vi "Configure Module.vi"(8 "error in (no error)":errorcluster, 10 "IOV ref in":variant, 11 "9224 in":refnum<class "9224.lvclass">) -> (0 "error out":errorcluster, 2 "IOV ref out":variant, 3 "9224 out":refnum<class "9224.lvclass">)   [LabVIEW 2020, in "Modules.lvlib" / "9224.lvclass"]
uses:
  9224.lvclass
  <resource>/objmgr/cRIO.rc
  RSI Module/RSI Module.lvclass
  C:/Users/nitest/Desktop/Git 2020/niveristand-scan-engine-module-libraries/Source/RSI Module/RSI Module.lvclass
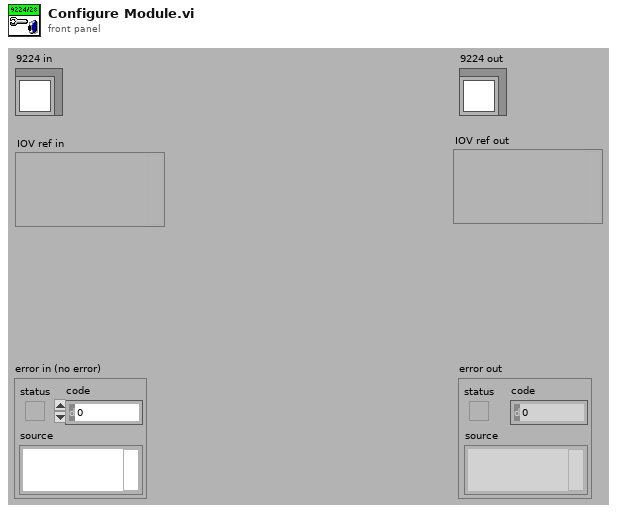
[diagram p1: front panel]
types:
  T1 = typedef "Modules.lvlib/9224.lvclass/Conversion Time.ctl" = u16
  T2 = typedef "Modules.lvlib/RSI Module.lvclass/Module Models.ctl" = enum16{"Empty", "NI 9201", "NI 9203", "NI 9205", "NI 9206", "NI 9207", "NI 9208", "NI 9209", "NI 9210", "NI 9211", "NI 9212", "NI 9213", "NI 9214", "NI 9215", "NI 9216", "NI 9217", "NI 9219", "NI 9220", "NI 9221", "NI 9222", "NI 9223", "NI 9224", "NI 9225", "NI 9226", "NI 9227", "NI 9228", "NI 9229", "NI 9233", "NI 9234", "NI 9235", "NI 9236", "NI 9237", "NI 9239", "NI 9242", "NI 9244", "NI 9253", "NI 9263", "NI 9264", "NI 9265", "NI 9266", "NI 9269", "NI 9344", "NI 9350", "NI 9375", "NI 9401", "NI 9402", "NI 9403", "NI 9411", "NI 9421", "NI 9422", "NI 9423", "NI 9425", "NI 9426", "NI 9435", "NI 9436", "NI 9437", "NI 9472", "NI 9474", "NI 9475", "NI 9476", "NI 9477", "NI 9478", "NI 9481", "NI 9482", "NI 9485"}
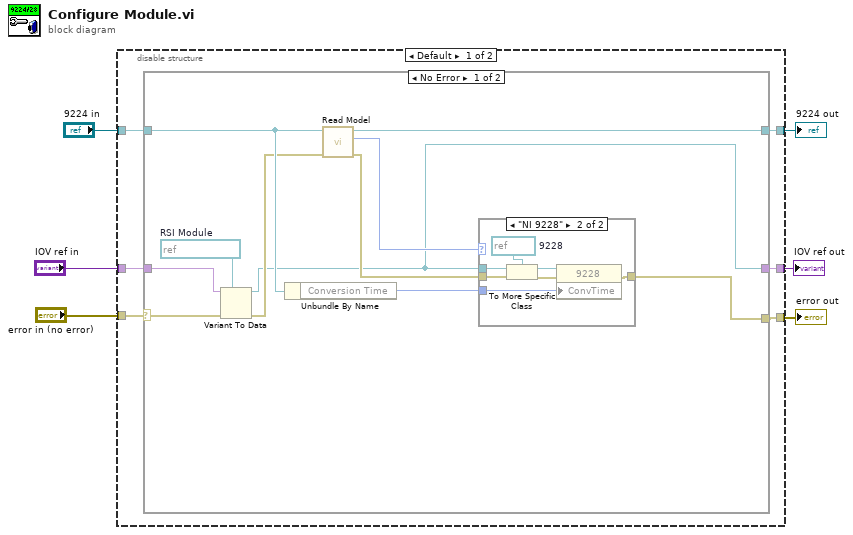
[diagram p0: block diagram]
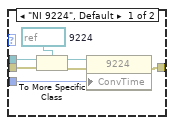
[diagram p2: hidden frame]
diagram:
  n1 = disable-structure shown="Default" {
    disable-tunnel: "9224 in" -> [w12 w43]
    disable-tunnel: "IOV ref in" -> [w11 w42]
    disable-tunnel: "error in (no error)" -> [w10 w41]
    disable-tunnel: [w9 w41] -> w3
    disable-tunnel: [w8 w42] -> w2
    disable-tunnel: [w7 w43] -> w1
    frame condition #0 {
      n2 = case shown="No Error" w10 {
        selector: w10 -> [w22 w40]
        tunnel: [w17 w40] -> w9
        tunnel: [w23 w39] -> w7
        tunnel: w12 -> [w21 w39]
        tunnel: w11 -> [w15 w38]
        tunnel: [w14 w38] -> w8
        frame No Error {
          w13 = refnum<k21> refnum  # RSI Module
          n3 = Variant To Data(error in=w22, type=w13, Variant=w15) -> (data=w14:refnum<k21>, error out=w16:errorcluster)
          n4 = Unbundle By Name(w21) -> ("Conversion Time"=w18:T1)
          n5 = call "Read Model.vi"("error in (no error)"=w16, "RSI Module in"=w21) -> ("error out"=w19:errorcluster, "Model"=w20:T2, "RSI Module out"=w23:refnum<class "9224.lvclass">)  [unwired: 7 in]
          n6 = case shown="\"NI 9228\"" w20 {
            tunnel: w19 -> [w30 w31]
            tunnel: [w26 w32] -> w17
            tunnel: w14 -> [w25 w33]
            tunnel: w18 -> [w24 w35]
            frame "NI 9224", Default {
              w29 = refnum<k21> refnum  # 9224
              n7 = To More Specific Class(target class=w29, reference=w25, error in=w30) -> (specific class reference=w28:refnum<k21>, error out=w27:errorcluster)
              n8 = property class="9224"(reference=w28, error in=w27, "ConvTime"=w24) -> (error out=w26:errorcluster)  [unwired: 1 out]
            }
            frame "NI 9228" {
              w34 = refnum<k21> refnum  # 9228
              n9 = To More Specific Class(target class=w34, reference=w33, error in=w31) -> (specific class reference=w37:refnum<k21>, error out=w36:errorcluster)
              n10 = property class="9228"(reference=w37, error in=w36, "ConvTime"=w35) -> (error out=w32:errorcluster)  [unwired: 1 out]
            }
          }
        }
        frame Error {
        }
      }
    }
    frame condition #1 (active) {
    }
  }
  "error out" <- w3
  "9224 out" <- w1
  "IOV ref out" <- w2
